vi "VIH Project - New Project - Master Rule (Default).vi"(8 "error in":errorcluster) -> (0 "error out":errorcluster, 3 "Master Rule":T1)   [LabVIEW 2014]
doc: "::: VI Helpeks :::\nCopyright (c) 2000-2026 Konstantin Shifershteyn. All rights reserved."
uses:
  _VIH HelpGen.llb/VIH HelpGen Typedef - Cluster - Group Rule.ctl
  _VIH HelpGen.llb/VIH HelpGen Typedef - Enum - Default,Enable,Disable.ctl
  _VIH HelpGen.llb/VIH HelpGen Typedef - Cluster - Group Rule - Source Paths.ctl
  _VIH HelpGen.llb/VIH HelpGen Typedef - Cluster - Group Rule - Target Paths.ctl
  _VIH HelpGen.llb/VIH HelpGen Typedef - Enum - Description Mode.ctl
  _VIH HelpGen.llb/VIH HelpGen Typedef - Cluster - Control Rule.ctl
  _VIH HelpGen.llb/VIH HelpGen Typedef - Cluster - Enum Value Info.ctl
  _VIH HelpGen.llb/VIH HelpGen Typedef - Cluster - Group Rule - Flags.ctl
panel:
  # "VI Helpeks\nCopyright (c) 2012-2026 Konstantin Shifershteyn"
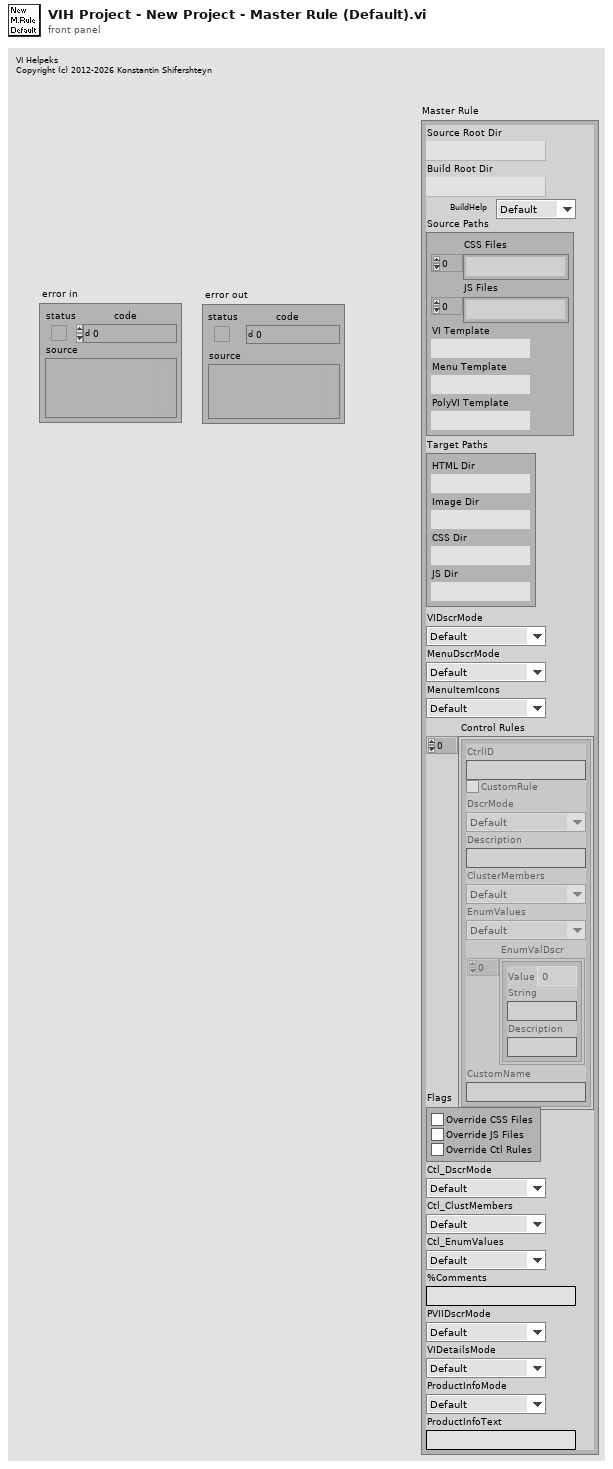
[diagram p1: front panel]
types:
  T1 = typedef "VIH HelpGen Typedef - Cluster - Group Rule.ctl" = cluster{"Source Root Dir":path, "Build Root Dir":path, "BuildHelp":T2, "Source Paths":T3, "Target Paths":T4, "VIDscrMode":T5, "MenuDscrMode":T5, "MenuItemIcons":T2, "Control Rules":T6[], "Flags":T8, "Ctl_DscrMode":T5, "Ctl_ClustMembers":T2, "Ctl_EnumValues":T2, "%Comments":string, "PVIIDscrMode":T5, "VIDetailsMode":T5, "ProductInfoMode":T2, "ProductInfoText":string}
  T2 = typedef "VIH HelpGen Typedef - Enum - Default,Enable,Disable.ctl" = enum16{"Default", "Enable", "Disable"}
  T3 = typedef "VIH HelpGen Typedef - Cluster - Group Rule - Source Paths.ctl" = cluster{"CSS Files":path[], "JS Files":path[], "VI Template":path, "Menu Template":path, "PolyVI Template":path}
  T4 = typedef "VIH HelpGen Typedef - Cluster - Group Rule - Target Paths.ctl" = cluster{"HTML Dir":path, "Image Dir":path, "CSS Dir":path, "JS Dir":path}
  T5 = typedef "VIH HelpGen Typedef - Enum - Description Mode.ctl" = enum16{"Default", "Description", "Description1", "Description2", "Custom", "None"}
  T6 = typedef "VIH HelpGen Typedef - Cluster - Control Rule.ctl" = cluster{"CtrlID":string, "CustomRule":bool, "DscrMode":T5, "Description":string, "ClusterMembers":T2, "EnumValues":T2, "EnumValDscr":T7[], "CustomName":string}
  T7 = typedef "VIH HelpGen Typedef - Cluster - Enum Value Info.ctl" = cluster{"Value":ext, "String":string, "Description":string}
  T8 = typedef "VIH HelpGen Typedef - Cluster - Group Rule - Flags.ctl" = cluster{"Override CSS Files":bool, "Override JS Files":bool, "Override Ctl Rules":bool}
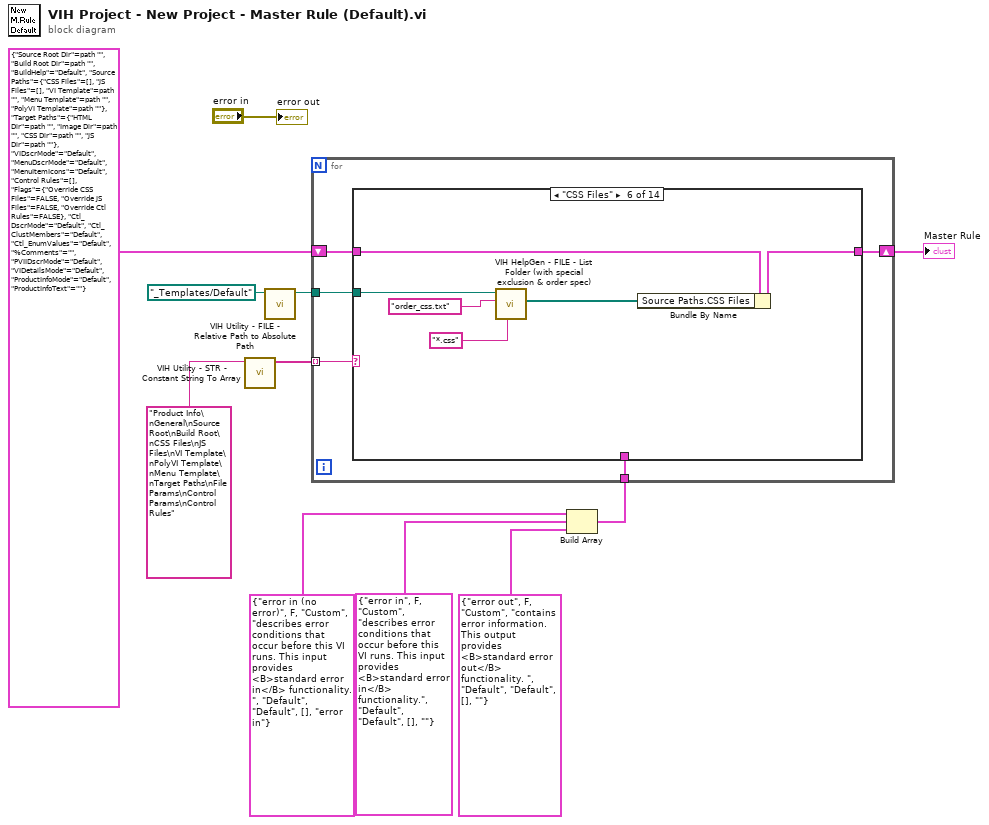
[diagram p0: block diagram]
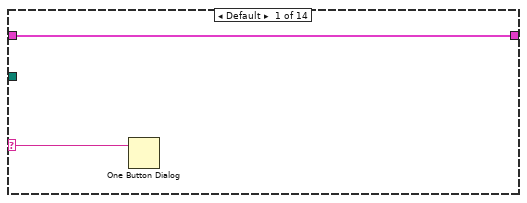
[diagram p2: hidden frame]
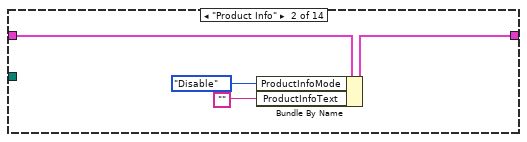
[diagram p3: hidden frame]
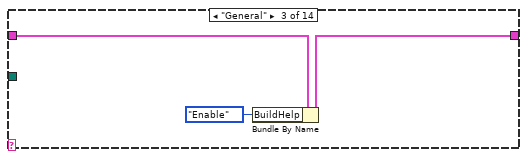
[diagram p4: hidden frame]
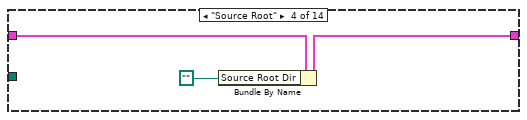
[diagram p5: hidden frame]
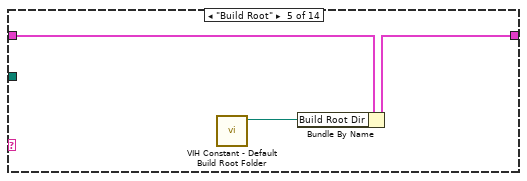
[diagram p6: hidden frame]
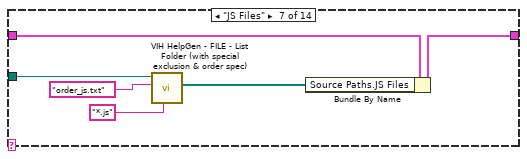
[diagram p7: hidden frame]
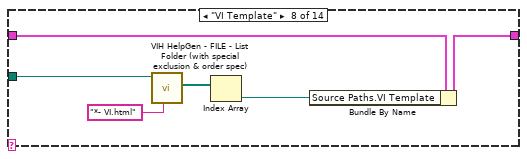
[diagram p8: hidden frame]
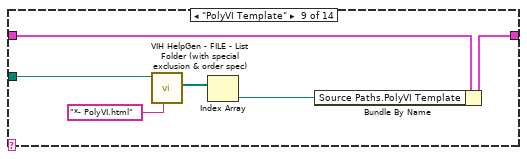
[diagram p9: hidden frame]
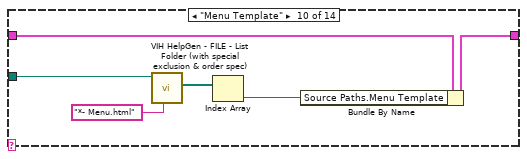
[diagram p10: hidden frame]
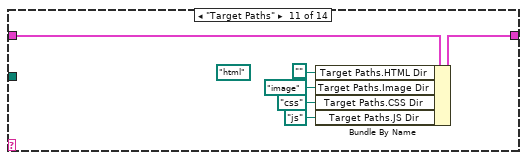
[diagram p11: hidden frame]
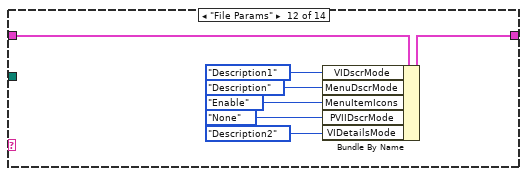
[diagram p12: hidden frame]
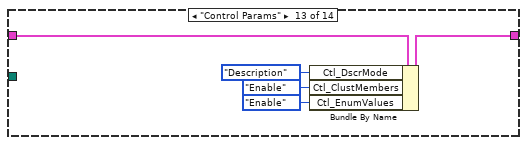
[diagram p13: hidden frame]
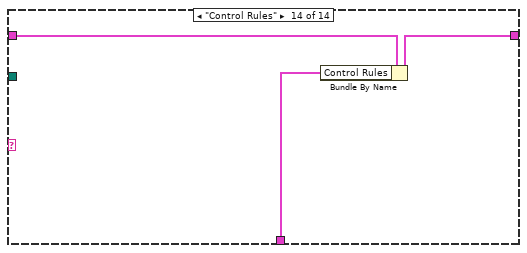
[diagram p14: hidden frame]
diagram:
  n1 = call "VIH Utility - STR - Constant String To Array.vi"("String in"="Product Info\nGeneral\nSource Root\nBuild Root\nCSS Files\nJS Files\nVI Template\nPolyVI Template\nMenu Template\nTarget Paths\nFile Params\nControl Params\nControl Rules") -> ("Array out"=w5:string[])  [unwired: 10 in]
  n2 = call "VIH Utility - FILE - Relative Path to Absolute Path.vi"("Path"=path "_Templates/Default") -> ("Path out"=w2:path)  [unwired: 9 in, 1 out]
  n3 = Build Array(T6 {"CtrlID"="error in (no error)", "CustomRule"=FALSE, "DscrMode"=enum."Custom", "Description"="describes error conditions that occur before this VI runs. This input provides <B>standard error in</B> functionality.", "ClusterMembers"=enum."Default", "EnumValues"=enum."Default", "EnumValDscr"=[], "CustomName"="error in"} ("Control Rule"), T6 {"CtrlID"="error in", "CustomRule"=FALSE, "DscrMode"=enum."Custom", "Description"="describes error conditions that occur before this VI runs. This input provides <B>standard error in</B> functionality.", "ClusterMembers"=enum."Default", "EnumValues"=enum."Default", "EnumValDscr"=[], "CustomName"=""} ("Control Rule"), T6 {"CtrlID"="error out", "CustomRule"=FALSE, "DscrMode"=enum."Custom", "Description"="contains error information. This output provides <B>standard error out</B> functionality. ", "ClusterMembers"=enum."Default", "EnumValues"=enum."Default", "EnumValDscr"=[], "CustomName"=""} ("Control Rule")) -> (w7:T6[])
  n4 = for {
    shift-right: [w16] -> w1
    shift-left: T1 {"Source Root Dir"=path "", "Build Root Dir"=path "", "BuildHelp"=enum."Default", "Source Paths"={"CSS Files"=[], "JS Files"=[], "VI Template"=path "", "Menu Template"=path "", "PolyVI Template"=path ""}, "Target Paths"={"HTML Dir"=path "", "Image Dir"=path "", "CSS Dir"=path "", "JS Dir"=path ""}, "VIDscrMode"=enum."Default", "MenuDscrMode"=enum."Default", "MenuItemIcons"=enum."Default", "Control Rules"=[], "Flags"={"Override CSS Files"=FALSE, "Override JS Files"=FALSE, "Override Ctl Rules"=FALSE}, "Ctl_DscrMode"=enum."Default", "Ctl_ClustMembers"=enum."Default", "Ctl_EnumValues"=enum."Default", "%Comments"="", "PVIIDscrMode"=enum."Default", "VIDetailsMode"=enum."Default", "ProductInfoMode"=enum."Default", "ProductInfoText"=""} ("Rule out") -> [w15]
    tunnel: w5 -> [w14] mode=indexing
    tunnel: w7 -> [w13]
    tunnel: w2 -> [w12]
    n5 = case shown="\"CSS Files\"" w14 {
      selector: w14 -> [w17 _ _ _ _ _ _ _ _ _ _ _ _ _]
      tunnel: [w18 w22 w24 w27 w30 w37 w43 w49 w55 w61 w67 w74 w79 w82] -> w16
      tunnel: w15 -> [w18 w21 w25 w28 w31 w36 w42 w48 w54 w60 w66 w73 w78 w81]
      tunnel: w13 -> [_ _ _ _ _ _ _ _ _ _ _ _ _ w80]
      tunnel: w12 -> [_ _ _ _ _ w34 w40 w45 w51 w57 _ _ _ _]
      frame Default {
        n6 = One Button Dialog(message=w17) -> ()  [unwired: 1 in, 1 out]
      }
      frame "Product Info" {
        n7 = Bundle By Name(cluster=w21, "ProductInfoMode"=VIH_HelpGen_Typedef_-_Enum_-_Default,Enable,Disable."Disable", "ProductInfoText"="") -> (w22:T1)
      }
      frame "General" {
        n8 = Bundle By Name(cluster=w25, "BuildHelp"=VIH_HelpGen_Typedef_-_Enum_-_Default,Enable,Disable."Enable") -> (w24:T1)
      }
      frame "Source Root" {
        n9 = Bundle By Name(cluster=w28, "Source Root Dir"=path "") -> (w27:T1)
      }
      frame "Build Root" {
        n10 = call "VIH Constant - Default Build Root Folder.vi"() -> ("Default Build Root Folder"=w29:path)  [unwired: 11 in]
        n11 = Bundle By Name(cluster=w31, "Build Root Dir"=w29) -> (w30:T1)
      }
      frame "CSS Files" {
        n12 = call "VIH HelpGen - FILE - List Folder (with special exclusion & order spec).vi"("pattern"="*.css", "order file name"="order_css.txt", "path"=w34) -> ("File paths"=w33:path[])  [unwired: 6 in, 2 out]
        n13 = Bundle By Name(cluster=w36, "Source Paths.CSS Files"=w33) -> (w37:T1)
      }
      frame "JS Files" {
        n14 = call "VIH HelpGen - FILE - List Folder (with special exclusion & order spec).vi"("pattern"="*.js", "order file name"="order_js.txt", "path"=w40) -> ("File paths"=w39:path[])  [unwired: 6 in, 2 out]
        n15 = Bundle By Name(cluster=w42, "Source Paths.JS Files"=w39) -> (w43:T1)
      }
      frame "VI Template" {
        n16 = call "VIH HelpGen - FILE - List Folder (with special exclusion & order spec).vi"("pattern"="*- VI.html", "path"=w45) -> ("File paths"=w46:path[])  [unwired: 7 in, 2 out]
        n17 = Index Array(array=w46) -> (element=w44:path)  [unwired: 1 in]
        n18 = Bundle By Name(cluster=w48, "Source Paths.VI Template"=w44) -> (w49:T1)
      }
      frame "PolyVI Template" {
        n19 = call "VIH HelpGen - FILE - List Folder (with special exclusion & order spec).vi"("pattern"="*- PolyVI.html", "path"=w51) -> ("File paths"=w52:path[])  [unwired: 7 in, 2 out]
        n20 = Index Array(array=w52) -> (element=w50:path)  [unwired: 1 in]
        n21 = Bundle By Name(cluster=w54, "Source Paths.PolyVI Template"=w50) -> (w55:T1)
      }
      frame "Menu Template" {
        n22 = call "VIH HelpGen - FILE - List Folder (with special exclusion & order spec).vi"("pattern"="*- Menu.html", "path"=w57) -> ("File paths"=w58:path[])  [unwired: 7 in, 2 out]
        n23 = Index Array(array=w58) -> (element=w56:path)  [unwired: 1 in]
        n24 = Bundle By Name(cluster=w60, "Source Paths.Menu Template"=w56) -> (w61:T1)
      }
      frame "Target Paths" {
        (unwired) path "html" ("Target Paths.HTML Dir")
        n25 = Bundle By Name(cluster=w66, "Target Paths.HTML Dir"=path "", "Target Paths.Image Dir"=path "image", "Target Paths.CSS Dir"=path "css", "Target Paths.JS Dir"=path "js") -> (w67:T1)
      }
      frame "File Params" {
        n26 = Bundle By Name(cluster=w73, "VIDscrMode"=VIH_HelpGen_Typedef_-_Enum_-_Description_Mode."Description1", "MenuDscrMode"=VIH_HelpGen_Typedef_-_Enum_-_Description_Mode."Description", "MenuItemIcons"=VIH_HelpGen_Typedef_-_Enum_-_Default,Enable,Disable."Enable", "PVIIDscrMode"=VIH_HelpGen_Typedef_-_Enum_-_Description_Mode."None", "VIDetailsMode"=VIH_HelpGen_Typedef_-_Enum_-_Description_Mode."Description2") -> (w74:T1)
      }
      frame "Control Params" {
        n27 = Bundle By Name(cluster=w78, "Ctl_DscrMode"=VIH_HelpGen_Typedef_-_Enum_-_Description_Mode."Description", "Ctl_ClustMembers"=VIH_HelpGen_Typedef_-_Enum_-_Default,Enable,Disable."Enable", "Ctl_EnumValues"=VIH_HelpGen_Typedef_-_Enum_-_Default,Enable,Disable."Enable") -> (w79:T1)
      }
      frame "Control Rules" {
        n28 = Bundle By Name(cluster=w81, "Control Rules"=w80) -> (w82:T1)
      }
    }
  }
  "Master Rule" <- w1
  "error out" <- "error in"
